vi "Test MQTT-2.3.1-6.vi"(8 "error in (no error)":errorcluster, 11 "Connection Config":refnum<class "Connection.lvclass">) -> (0 "error out":errorcluster, 3 "Connection Config dup":refnum<class "Connection.lvclass">)   [LabVIEW 2013]
uses:
  <vilib>/LabVIEW Open Source Project/MQTT Connection/MQTT_Connection/Connection/Connection.lvclass
  <vilib>/LabVIEW Open Source Project/MQTT Control Packets/Control Packets/ControlPacket/QualityOfService -- enum.ctl
  <vilib>/addons/_JKI Toolkits/Caraya/classes/Test/Test.lvclass
  <vilib>/addons/_JKI Toolkits/Caraya/classes/Assert/Assert.lvclass
  <vilib>/LabVIEW Open Source Project/MQTT Client/Client class/Client.lvclass
  <vilib>/LabVIEW Open Source Project/MQTT Control Packets/Control Packets/ControlPacket/ControlPacket.lvclass
  <vilib>/LabVIEW Open Source Project/MQTT Connection/MQTT_Base/Base Class/MQTT_Base.lvclass
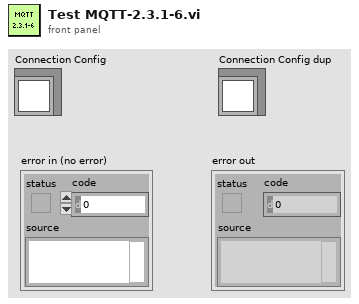
[diagram p1: front panel]
types:
  T1 = typedef "MQTT_Control_Packets.lvlib/ControlPacket.lvclass/QualityOfService -- enum.ctl" = enum16{"0 (At Most Once)", "1 (At Least Once)", "2 (Exactly Once)"}
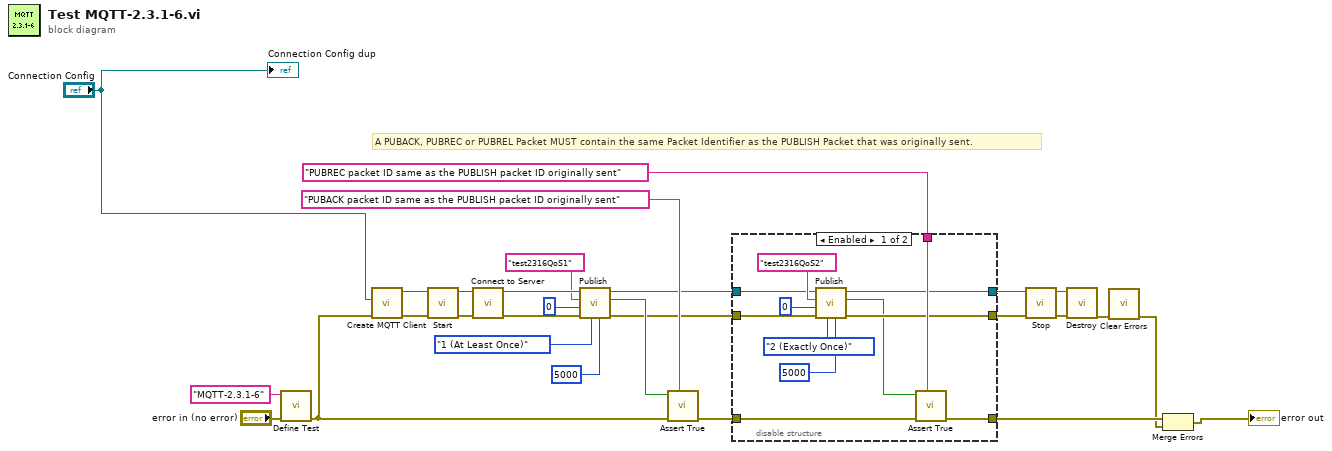
[diagram p0: block diagram]
diagram:
  # "A PUBACK, PUBREC or PUBREL Packet MUST contain the same Packet Identifier as the PUBLISH Packet that was originally sent."
  n1 = call <vilib>:"Define Test.vi"("error in (no error)"="error in (no error)", "Label (VI Title)"="MQTT-2.3.1-6") -> ("error out"=w25:errorcluster)  [unwired: 9 in]
  n2 = call <vilib>:"Create MQTT Client.vi"("error in (no error)"=w25, "Connection Configuration"="Connection Config") -> ("error out"=w20:errorcluster, "Client out"=w21:refnum<class "Client.lvclass">)  [unwired: 8 in]
  n3 = call <vilib>:"Start.vi"("error in (no error)"=w20, "MQTT_Base in"=w21) -> ("error out"=w23:errorcluster, "MQTT_Base out"=w24:refnum<class "Client.lvclass">)  [unwired: 7 in, 1 out]
  n4 = call <vilib>:"Connect to Server.vi"("error in (no error)"=w23, "Client in"=w24) -> ("error out"=w15:errorcluster, "Client out"=w16:refnum<class "Client.lvclass">)  [unwired: 6 in, 2 out]
  n5 = call <vilib>:"Publish.vi"("timeout (1000ms)"=5000, "QoS"=QualityOfService_--_enum."1 (At Least Once)", "error in (no error)"=w15, "Payload"=0, "Topic Name (empty: Payload name)"="test2316QoS1", "Client in"=w16) -> ("error out"=w6:errorcluster, "Published"=w11:bool, "Client out"=w7:refnum<class "Client.lvclass">)  [unwired: 3 in]
  n6 = call <vilib>:"Assert True.vi"("Label"="PUBACK packet ID same as the PUBLISH packet ID originally sent", "error in (no error)"=w25, "True?"=w11) -> ("error out"=w10:errorcluster)  [unwired: 8 in]
  n7 = disable-structure "Diagram Disable Structure" shown="Enabled" {
    disable-tunnel: w10 -> [w40 w41]
    disable-tunnel: [w39 w41] -> w9
    disable-tunnel: "PUBREC packet ID same as the PUBLISH packet ID originally sent" ("Label") -> [w38 _]
    disable-tunnel: w7 -> [w34 w43]
    disable-tunnel: w6 -> [w33 w42]
    disable-tunnel: [w32 w43] -> w5
    disable-tunnel: [w31 w42] -> w4
    frame Enabled {
      n8 = call <vilib>:"Publish.vi"("timeout (1000ms)"=5000, "QoS"=QualityOfService_--_enum."2 (Exactly Once)", "error in (no error)"=w33, "Payload"=0, "Topic Name (empty: Payload name)"="test2316QoS2", "Client in"=w34) -> ("error out"=w31:errorcluster, "Published"=w30:bool, "Client out"=w32:refnum<class "Client.lvclass">)  [unwired: 3 in]
      n9 = call <vilib>:"Assert True.vi"("Label"=w38, "error in (no error)"=w40, "True?"=w30) -> ("error out"=w39:errorcluster)  [unwired: 8 in]
    }
    frame Disabled {
    }
  }
  n10 = call <vilib>:"Stop.vi"("error in (no error)"=w4, "MQTT_Base in"=w5) -> ("error out"=w17:errorcluster, "MQTT_Base out"=w22:refnum<class "Client.lvclass">)  [unwired: 7 in, 1 out]
  n11 = call <vilib>:"Destroy.vi"("error in (no error)"=w17, "MQTT_Base in"=w22) -> ("error out"=w19:errorcluster)  [unwired: 8 in, 1 out]
  n12 = call <vilib>:"Clear Errors.vi"("error in (no error)"=w19) -> ("error out"=w1:errorcluster)  [unwired: 6 in]
  n13 = Merge Errors(w9, w1) -> (→"error out":errorcluster)
  "Connection Config dup" <- "Connection Config"
